vi "Loop Probe.vi"(0 "N":i32=5) -> (1 "Count":i32)   [LabVIEW 2026]
doc: "Round17 dialect-validation probe: a While Loop with one shift register that counts iterations until it reaches N. Validates the While Loop + ShiftReg + Condition + Tunnel AIXML dialect through the pylabview backend (no gRPC/Nigel). Expected: Count == N for N>=1 (Count=5 when N=5). Lesson: a constant feeding a loop-internal node must enter via a Tunnel; a constant feeding a shift-register terminal (at the loop boundary) must come from the root diagram (LV012)."
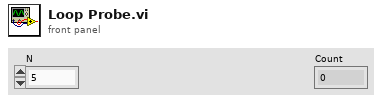
[diagram p1: front panel]
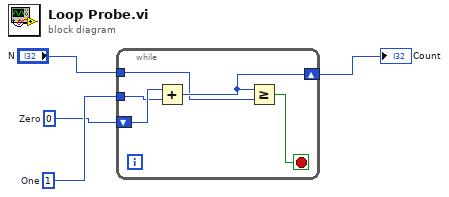
[diagram p0: block diagram]
diagram:
  w3 = 1  # One
  w2 = 0  # Zero
  n1 = while {
    tunnel: "N" -> [w5]
    tunnel: w3 -> [w6]
    shift-right: [w8] -> w4
    shift-left: w2 -> [w7]
    stop <- w9 stop-if-true
    n2 = Add(x=w7, y=w6) -> (x+y=w8:i32)
    n3 = Greater Or Equal?(x=w8, y=w5) -> (x >= y?=w9:bool)
  }
  "Count" <- w4
